vi "libssh2_sftp_close_handle.vi"(8 "error in (no error)":errorcluster, 11 "sftp handle":T1) -> (0 "error out":errorcluster)   [LabVIEW 2017, in "libssh2.lvlib"]
doc: "Close a file handle."
uses:
  libssh2.lvlib
  SFTP Handle Refnum.ctl
  Acquire Session.vi
  Release Session.vi
  Global Settings.vi
  Read SFTP Refnum.vi
  Read Session Refnum.vi
  <vilib>/Utility/semaphor.llb/Acquire Semaphore.vi
  <vilib>/Utility/semaphor.llb/Release Semaphore.vi
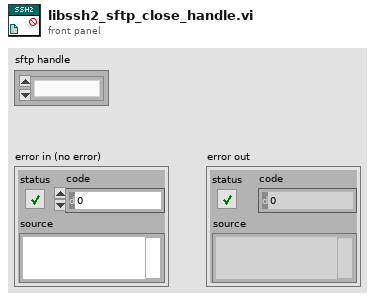
[diagram p1: front panel]
types:
  T1 = typedef "libssh2.lvlib/SFTP Handle Refnum.ctl" = refnum<k1>
  T2 = typedef "libssh2.lvlib/SFTP Refnum.ctl" = refnum<k1>
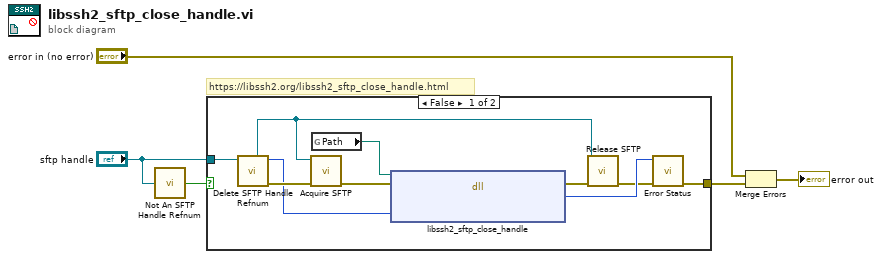
[diagram p0: block diagram]
diagram:
  # "https://libssh2.org/libssh2_sftp_close_handle.html"
  n1 = call "Not An SFTP Handle Refnum.vi"("sftp handle"="sftp handle") -> ("Not a SFTP Handle Refnum?"=w5:bool)
  n2 = case shown="False" w5 {
    tunnel: "sftp handle" -> [w14 _]
    tunnel: [w10 _] -> w4
    frame False {
      n3 = call "Delete SFTP Handle Refnum.vi"("sftp handle"=w14) -> ("error out"=w13:errorcluster, "LIBSSH2_SFTP_HANDLE*"=w12:u64, "sftp"=w6:T2)  [unwired: 8 in]
      n4 = call "Acquire SFTP.vi"("error in (no error)"=w13, "sftp"=w6) -> ("error out"=w8:errorcluster)  [unwired: 8 in, 1 out]
      n5 = global read "Global Settings.vi" "Path"() -> (w15:path)
      n6 = dll-call lib="?" fn="libssh2_sftp_close_handle"(path in=w15, error in=w8, "handle"=w12) -> (error out=w11:errorcluster, "return value"=w9:i32)  [unwired: 2 in, 1 out]
      n7 = call "Release SFTP.vi"("error in (no error)"=w11, "sftp"=w6) -> ("error out"=w7:errorcluster)  [unwired: 9 in]
      n8 = call "Error Status.vi"("error in (no error)"=w7, "return value"=w9) -> ("error out"=w10:errorcluster)  [unwired: 8 in, 1 out]
    }
    frame True {
    }
  }
  n9 = Merge Errors("error in (no error)", w4) -> (→"error out":errorcluster)
